vi "Filter.vi"(10 "file path":path, 11 "CleanupFilter in":refnum<class "CleanupFilter.lvclass">) -> (2 "cleanup?":bool, 3 "CleanupFilter out":refnum<class "CleanupFilter.lvclass">)   [LabVIEW 2018, in "GLog.lvlib" / "CleanupFilter.lvclass"]
uses:
  CleanupFilter.lvclass
  73983668-8d2c-423d-9a11-a3a53d6b3ce1.vi
panel:
  # "Connector Pane"
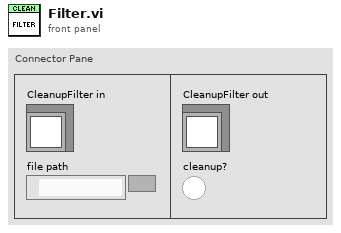
[diagram p1: front panel]
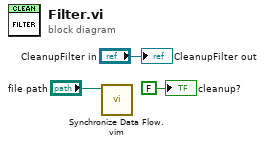
[diagram p0: block diagram]
diagram:
  n1 = call "Synchronize Data Flow.vim"("input 1"="file path") -> ()  [unwired: 3 in, 4 out]
  "CleanupFilter out" <- "CleanupFilter in"
  "cleanup?" <- FALSE ("cleanup?")
